vi "Get Variant structure.vi"(10 "variant in":variant) -> (2 "<JSON>":string)   [LabVIEW 2020, in "LabVIEW-Python TCP Lib.lvlib"]
uses:
  LabVIEW-Python TCP Lib.lvlib
  <vilib>/JDP Science/JSONtext/JSONtext.lvlib
  <vilib>/Utility/Data Type/NI_Data Type.lvlib
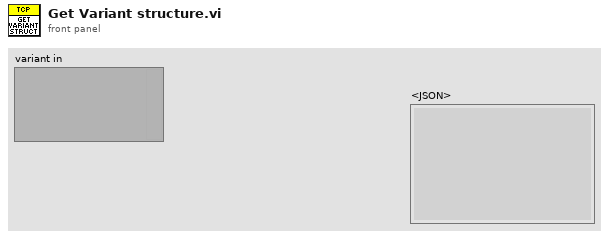
[diagram p1: front panel]
types:
  T1 = typedef "NI_Data Type.lvlib/Data Type.ctl" = enum8{"Invalid Type", "Void", "I8", "I16", "I32", "I64", "U8", "U16", "U32", "U64", "Single Float", "Double Float", "Extended Float", "Single Complex", "Double Complex", "Extended Complex", "Enum U8", "Enum U16", "Enum U32", "Enum U64", "Single Float With Unit", "Double Float With Unit", "Extended Float With Unit", "Single Complex with Unit", "Double Complex with Unit", "Extended Complex with Unit", "Boolean", "String", "Path", "Picture", "Tag", "Array", "Cluster", "Variant", "LV Variant", "Waveform", "Timestamp", "Digital Waveform", "Digital Data", "ExpressData", "Refnum", "External Data", "VI", "Poly VI", "LabVIEW Class Instance", "Fixed Point", "Set Collection", "Map Collection"}
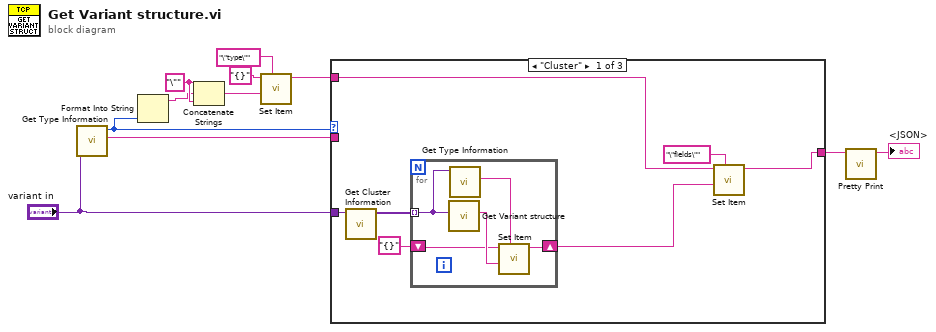
[diagram p0: block diagram]
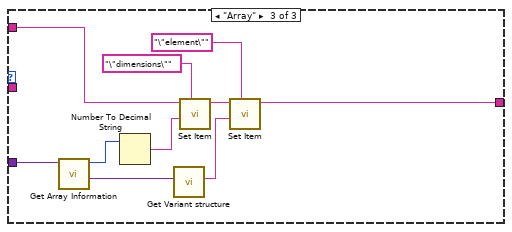
[diagram p3: hidden frame]
diagram:
  w7 = "\"" ("string")
  n1 = call <vilib>:"Get Type Information.vi"("variant"="variant in") -> ("name"=w11:string, "type"=w2:T1)  [unwired: 6 in, 3 out]
  n2 = Format Into String(w2) -> (resulting string=w1:string)  [unwired: 3 in, 1 out]
  n3 = Concatenate Strings(w7, w1, w7) -> (w4:string)
  n4 = call <vilib>:"Set Item.vi"("$Path or Item Name"="\"type\"", "JSON to Insert"=w4, "JSON"="{}") -> ("<JSON>"=w3:string)  [unwired: 5 in, 2 out]
  n5 = case shown="\"Cluster\"" w2 {
    tunnel: [w12 w24 w26] -> w9
    tunnel: w11 -> [_ _ _]
    tunnel: "variant in" -> [w17 _ w34]
    tunnel: w3 -> [w13 w24 w25]
    frame "Cluster" {
      n6 = call <vilib>:"Get Cluster Information.vi"("variant"=w17) -> ("cluster elements"=w18:variant[])  [unwired: 9 in, 1 out]
      n7 = for {
        tunnel: w18 -> [w23] mode=indexing
        shift-right: [w20] -> w15
        shift-left: "{}" ("<JSON>") -> [w19]
        n8 = call "Get Variant structure.vi"("variant in"=w23) -> ("<JSON>"=w21:string)  [unwired: 10 in]
        n9 = call <vilib>:"Get Type Information.vi"("variant"=w23) -> ("name"=w22:string)  [unwired: 6 in, 4 out]
        n10 = call <vilib>:"Set Item.vi"("$Path or Item Name"=w22, "JSON to Insert"=w21, "JSON"=w19) -> ("<JSON>"=w20:string)  [unwired: 5 in, 2 out]
      }
      n11 = call <vilib>:"Set Item.vi"("$Path or Item Name"="\"fields\"", "JSON to Insert"=w15, "JSON"=w13) -> ("<JSON>"=w12:string)  [unwired: 5 in, 2 out]
    }
    frame Default {
    }
    frame "Array" {
      n12 = call <vilib>:"Get Array Information.vi"("variant"=w34) -> ("array element data type"=w33:variant, "number of dimensions"=w32:i32)  [unwired: 7 in, 2 out]
      n13 = Number To Decimal String(number=w32) -> (decimal integer string=w31:string)  [unwired: 1 in]
      n14 = call "Get Variant structure.vi"("variant in"=w33) -> ("<JSON>"=w28:string)  [unwired: 10 in]
      n15 = call <vilib>:"Set Item.vi"("$Path or Item Name"="\"dimensions\"", "JSON to Insert"=w31, "JSON"=w25) -> ("<JSON>"=w27:string)  [unwired: 5 in, 2 out]
      n16 = call <vilib>:"Set Item.vi"("$Path or Item Name"="\"element\"", "JSON to Insert"=w28, "JSON"=w27) -> ("<JSON>"=w26:string)  [unwired: 5 in, 2 out]
    }
  }
  n17 = call <vilib>:"Pretty Print.vi"("JSON"=w9) -> ("<JSON>"=→"<JSON>":string)  [unwired: 8 in, 2 out]
